vi "RemoteVI Check Translate Input.vi"() -> (4 "labels":string[](array[string]), 6 "expected":string[](array[string]), 8 "actual":string[](array[string]), 10 "failures":i32)   [LabVIEW 2020]
doc: "Test support, generated by tests/caraya/build.py from tests/vectors/translate.json (cases) - do not edit. Calls RemoteVI Translate Input.vi once per vector: the vector's input text goes through RemoteVI Parse Input.vi first, geo is the vector's geo, tracking in is trackingBefore; posts are rendered msg:wParam:lParam; each, cursor as x,y or - when the vector's cursor is null (move? FALSE). Outputs, one element per vector: labels (the vector's name), expected (rendered from the vector), actual (the VI's result rendered the same way), and failures, the number of vectors whose expected and actual differ."
uses:
  source/RemoteVI.lvlib
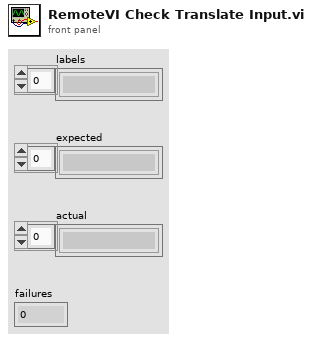
[diagram p1: front panel]
types:
  T1 = cluster{"name":string, "input":string, "popup":bool, "trackingBefore":bool, "expect":string}[]
  T2 = cluster{"panelX":i32, "panelY":i32, "clientX":i32, "clientY":i32}
  T3 = enum16{"invalid", "mouse", "key", "ack", "close", "splitter"}
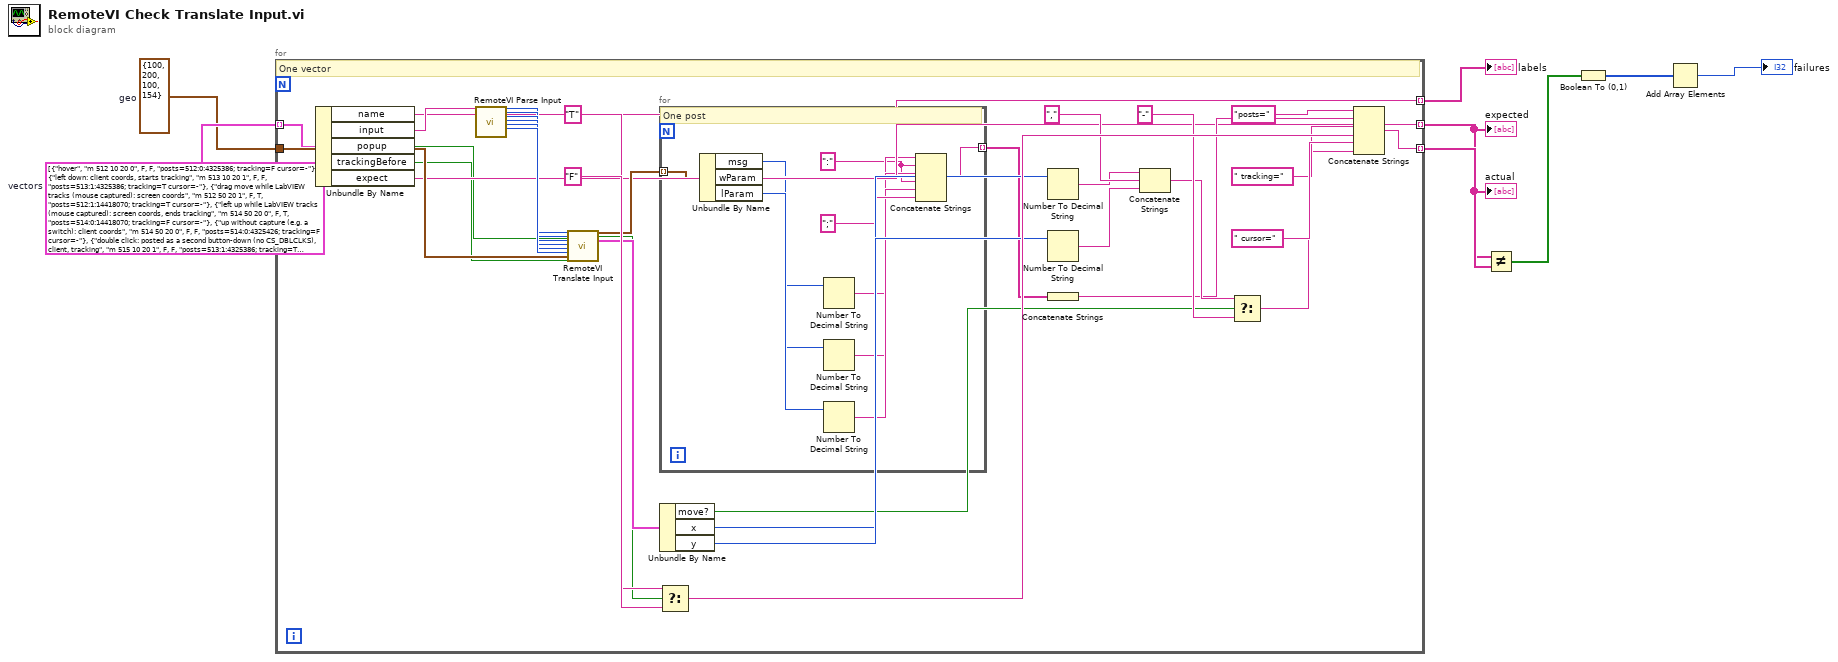
[diagram p0: block diagram]
diagram:
  w2 = T1 [{"name"="hover", "input"="m 512 10 20 0", "popup"=FALSE, "trackingBefore"=FALSE, "expect"="posts=512:0:4325386; tracking=F cursor=-"}, {"name"="left down: client coords, starts tracking", "input"="m 513 10 20 1", "popup"=FALSE, "trackingBefore"=FALSE, "expect"="posts=513:1:4325386; tracking=T cursor=-"}, {"name"="drag move while LabVIEW tracks (mouse captured): screen coords", "input"="m 512 50 20 1", "popup"=FALSE, "trackingBefore"=TRUE, "expect"="posts=512:1:14418070; tracking=T cursor=-"}, {"name"="left up while LabVIEW tracks (mouse captured): screen coords, ends tracking", "input"="m 514 50 20 0", "popup"=FALSE, "trackingBefore"=TRUE, "expect"="posts=514:0:14418070; tracking=F cursor=-"}, {"name"="up without capture (e.g. a switch): client coords", "input"="m 514 50 20 0", "popup"=FALSE, "trackingBefore"=FALSE, "expect"="posts=514:0:4325426; tracking=F cursor=-"}, {"name"="double click: posted as a second button-down (no CS_DBLCLKS), client, tracking", "input"="m 515 10 20 1", "popup"=FALSE, "trackingBefore"=FALSE, "expect"="posts=513:1:4325386; tracking=T cursor=-"}, {"name"="right double click: posted as a right button-down", "input"="m 518 5 5 2", "popup"=FALSE, "trackingBefore"=FALSE, "expect"="posts=516:2:3342341; tracking=T cursor=-"}, {"name"="right down", "input"="m 516 5 5 2", "popup"=FALSE, "trackingBefore"=FALSE, "expect"="posts=516:2:3342341; tracking=T cursor=-"}, {"name"="wheel: always screen coords", "input"="m 522 10 20 7864320", "popup"=FALSE, "trackingBefore"=FALSE, "expect"="posts=522:7864320:14418030; tracking=F cursor=-"}, {"name"="wheel while tracking", "input"="m 522 10 20 7864320", "popup"=FALSE, "trackingBefore"=TRUE, "expect"="posts=522:7864320:14418030; tracking=T cursor=-"}, {"name"="negative client y (toolbar area)", "input"="m 512 0 0 0", "popup"=FALSE, "trackingBefore"=FALSE, "expect"="posts=512:0:3014656; tracking=F cursor=-"}, {"name"="char is wrapped in VK 0xE8 down/up", "input"="k 258 65 1", "popup"=FALSE, "trackingBefore"=FALSE, "expect"="posts=256:232:1;258:65:1;257:232:3221225473; tracking=F cursor=-"}, {"name"="special key gets its scan code", "input"="k 256 13 1", "popup"=FALSE, "trackingBefore"=FALSE, "expect"="posts=256:13:1835009; tracking=F cursor=-"}, {"name"="key up gets its scan code, extended and up bits kept", "input"="k 257 37 3238002689", "popup"=FALSE, "trackingBefore"=FALSE, "expect"="posts=257:37:3242917889; tracking=F cursor=-"}, {"name"="extended key down (Right) gets its scan code", "input"="k 256 39 16777217", "popup"=FALSE, "trackingBefore"=FALSE, "expect"="posts=256:39:21823489; tracking=F cursor=-"}, {"name"="Shift down gets its scan code", "input"="k 256 16 1", "popup"=FALSE, "trackingBefore"=FALSE, "expect"="posts=256:16:2752513; tracking=F cursor=-"}, {"name"="a scan code the client sent is kept", "input"="k 256 13 1835009", "popup"=FALSE, "trackingBefore"=FALSE, "expect"="posts=256:13:1835009; tracking=F cursor=-"}, {"name"="key without a known scan code passes through", "input"="k 256 65 1", "popup"=FALSE, "trackingBefore"=FALSE, "expect"="posts=256:65:1; tracking=F cursor=-"}, {"name"="negative (signed) key-up lParam gets its scan code", "input"="k 257 13 -1073741823", "popup"=FALSE, "trackingBefore"=FALSE, "expect"="posts=257:13:-1071906815; tracking=F cursor=-"}, {"name"="not allowed: WM_CLOSE", "input"="m 16 1 1 0", "popup"=FALSE, "trackingBefore"=FALSE, "expect"="posts= tracking=F cursor=-"}, {"name"="not allowed: WM_SYSKEYDOWN", "input"="k 260 18 1", "popup"=FALSE, "trackingBefore"=FALSE, "expect"="posts= tracking=F cursor=-"}, {"name"="ack: nothing to post", "input"="a 5", "popup"=FALSE, "trackingBefore"=FALSE, "expect"="posts= tracking=F cursor=-"}, {"name"="popup open: moves are dropped (host cursor stays put)", "input"="m 512 10 20 0", "popup"=TRUE, "trackingBefore"=FALSE, "expect"="posts= tracking=F cursor=-"}, {"name"="popup open: wheel is dropped", "input"="m 522 10 20 7864320", "popup"=TRUE, "trackingBefore"=FALSE, "expect"="posts= tracking=F cursor=-"}, {"name"="popup open: click outside the panel (negative coords) still maps", "input"="m 513 -30 600 1", "popup"=TRUE, "trackingBefore"=FALSE, "expect"="posts=513:1:52428870; tracking=T cursor=70,800"}, {"name"="popup open: down uses screen coords, cursor, tracking", "input"="m 513 10 20 1", "popup"=TRUE, "trackingBefore"=FALSE, "expect"="posts=513:1:14418030; tracking=T cursor=110,220"}, {"name"="popup open: up uses screen coords, cursor, ends tracking", "input"="m 514 10 20 0", "popup"=TRUE, "trackingBefore"=TRUE, "expect"="posts=514:0:14418030; tracking=F cursor=110,220"}, {"name"="popup open: double click is posted as a button-down", "input"="m 515 10 20 1", "popup"=TRUE, "trackingBefore"=FALSE, "expect"="posts=513:1:14418030; tracking=T cursor=110,220"}, {"name"="popup open: char still wrapped, no cursor move", "input"="k 258 65 1", "popup"=TRUE, "trackingBefore"=FALSE, "expect"="posts=256:232:1;258:65:1;257:232:3221225473; tracking=F cursor=-"}]  # vectors
  w1 = T2 {"panelX"=100, "panelY"=200, "clientX"=100, "clientY"=154}  # geo
  n1 = for {
    tunnel: w2 -> [w9] mode=indexing
    tunnel: w1 -> [w15]
    tunnel: [w10] -> w3 mode=indexing
    tunnel: [w14] -> w4 mode=indexing
    tunnel: [w42] -> w5 mode=indexing
    # "One vector"
    n2 = Unbundle By Name(w9) -> ("name"=w10:string, "input"=w11:string, "popup"=w12:bool, "trackingBefore"=w13:bool, "expect"=w14:string)
    n3 = call "RemoteVI Parse Input.vi"("text"=w11) -> ("kind"=w16:T3, "msg"=w17:u32, "x"=w18:i32, "y"=w19:i32, "wParam"=w20:u64, "lParam"=w21:i64)  [unwired: 19 in, 2 out]
    n4 = call "RemoteVI Translate Input.vi"("kind"=w16, "msg"=w17, "x"=w18, "y"=w19, "wParam"=w20, "lParam"=w21, "geo"=w15, "tracking in"=w13, "popup"=w12) -> ("posts"=w22:cluster{"msg":u32, "wParam":u64, "lParam":i64}[], "tracking out"=w23:bool, "cursor"=w24:cluster{"move?":bool, "x":i32, "y":i32})  [unwired: 16 in]
    n5 = for {
      tunnel: w22 -> [w43] mode=indexing
      tunnel: [w52] -> w25 mode=indexing
      w47 = ":"
      # "One post"
      n6 = Unbundle By Name(w43) -> ("msg"=w44:u32, "wParam"=w45:u64, "lParam"=w46:i64)
      n7 = Number To Decimal String(number=w44) -> (decimal integer string=w48:string)  [unwired: 1 in]
      n8 = Number To Decimal String(number=w45) -> (decimal integer string=w49:string)  [unwired: 1 in]
      n9 = Number To Decimal String(number=w46) -> (decimal integer string=w50:string)  [unwired: 1 in]
      n10 = Concatenate Strings(w48, w47, w49, w47, w50, ";") -> (w52:string)
    }
    n11 = Unbundle By Name(w24) -> ("move?"=w27:bool, "x"=w28:i32, "y"=w29:i32)
    n12 = Select(t="T", s=w23, f="F") -> (s? t:f=w40:string)
    n13 = Number To Decimal String(number=w28) -> (decimal integer string=w30:string)  [unwired: 1 in]
    n14 = Number To Decimal String(number=w29) -> (decimal integer string=w32:string)  [unwired: 1 in]
    n15 = Concatenate Strings(w25) -> (w26:string)
    n16 = Concatenate Strings(w30, ",", w32) -> (w33:string)
    n17 = Select(t=w33, s=w27, f="-") -> (s? t:f=w35:string)
    n18 = Concatenate Strings("posts=", w26, " tracking=", w40, " cursor=", w35) -> (w42:string)
  }
  "labels" <- w3
  "expected" <- w4
  "actual" <- w5
  n19 = Not Equal?(x=w4, y=w5) -> (x != y?=w6:bool[])
  n20 = Boolean To (0,1)(Boolean=w6) -> (0, 1=w7:i16[])
  n21 = Add Array Elements(numeric array=w7) -> (sum=→"failures":i16)
